vi "MQTT Client - Close.vi"(0 "MQTT session":T1, 11 "error in (no error)":errorcluster) -> (15 "error out":errorcluster)   [LabVIEW 2019, in "KoRE-MQTT.lvlib"]
doc: "<b>Description:</b> This VI closes the MQTT client session. It ensures that the session is properly terminated to free up resources and maintain network integrity. \n\n<b>Input Terminals:</b>\n- <b>MQTT session [0]</b>: Reference to the active MQTT session that is to be closed.\n\n\nCopyright (c) 2025 KoRElibs.com\nSPDX-License-Identifier: EUPL-1.2\n\nThis VI is licensed under the European Union Public License (EUPL) Version 1.2. You may use this VI unmodified in proprietary works. If you distribute a modified version of this file, the modified file must be released under the EUPL-1.2. Full license: https://joinup.ec.europa.eu/asset/eupl/eupl/1.2/"
uses:
  KoRE-MQTT.lvlib
  TypeDefs/MQTT Client Session.ctl
  Private/TypeDefs/MQTT Client Session - Data Value Reference.ctl
  TypeDefs/MQTT Client Session - Data.ctl
  TypeDefs/MQTT Property - Will.ctl
  TypeDefs/MQTT Property - CONNECT.ctl
  Private/TypeDefs/MQTT Subscription - Info.ctl
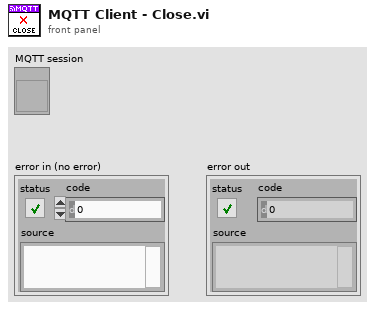
[diagram p1: front panel]
types:
  T1 = typedef "KoRE-MQTT.lvlib/MQTT Client Session.ctl" = refnum<vi>
  T2 = typedef "KoRE-MQTT.lvlib/MQTT Client Session - Data Value Reference.ctl" = refnum<data-value>
  T3 = typedef "KoRE-MQTT.lvlib/MQTT Client Session - Data.ctl" = cluster{"TCP ref":refnum<k5>, "Next Packet Id":u16, "Version":u8, "Host":string, "Port":u16, "Ping Delta":u32, "Username":string, "Password":string, "Will QoS":u8, "Will Retain":bool, "Will Topic":string, "Will Payload":string, "TCP Timeout":i32, "Semaphore":T4, "In-Flight Messages":variant, "Close":bool, "Last Send":u32, "Keep Alive":u16, "Last Ping RTT":u32, "Last Ping":u32, "Will Properties":T5[], "Session Expiry Interval":u32, "Maximum QoS":u8, "Retain Available":bool, "Server Maximum Packet Size":u32, "Client Identifier":string, "Server Topic Alias Maximum":u16, "Wildcard Subscription Available":bool, "Subscription Identifier Available":bool, "Shared Subscription Available":bool, "Connect Properties":T6[], "Client Maximum Packet Size":u32, "Client Topic Alias Maximum":u16, "Server Receive Maximum":u16, "Client Receive Maximum":u16, "TLS cfg":refnum<k36>, "Subscriptions":T7[]}
  T4 = typedef "Semaphore RefNum" = refnum<k1>
  T5 = typedef "KoRE-MQTT.lvlib/MQTT Property - Will.ctl" = cluster{"Property":u8, "Value":string}
  T6 = typedef "KoRE-MQTT.lvlib/MQTT Property - CONNECT.ctl" = cluster{"Property":u8, "Value":string}
  T7 = typedef "KoRE-MQTT.lvlib/MQTT Subscription - Info.ctl" = cluster{"Packet Id":u16, "Index":u16, "Identifier":u32, "QoS":u8, "Topic Filter":string, "Reason Code":u8, "Reason String":string, "Granted":bool}
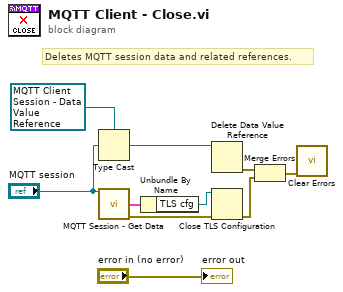
[diagram p0: block diagram]
diagram:
  # "Deletes MQTT session data and related references."
  n1 = Type Cast(type=T2 refnum ("data value reference"), x="MQTT session") -> (*(type *) &x=w10:T2)
  n2 = call "MQTT Session - Get Data.vi"("mqtt ref in"="MQTT session") -> ("mqtt ref data"=w7:T3, "error out"=w5:errorcluster)  [unwired: 12 in, 1 out]
  n3 = Unbundle By Name(w7) -> ("TLS cfg"=w6:refnum<k36>)
  n4 = Delete Data Value Reference(data value reference=w10) -> (error out=w4:errorcluster)  [unwired: 1 in, 1 out]
  n5 = Close TLS Configuration(8:w5, 11:w6) -> (0:w3:errorcluster)
  n6 = Merge Errors(w4, w3) -> (w2:errorcluster)
  n7 = call <vilib>:"Clear Errors.vi"("error in (no error)"=w2) -> ()  [unwired: 5 in, 2 out]
  "error out" <- "error in (no error)"
